vi "Event Handler.vi"(0 "Monkey in":refnum<class "Monkey.lvclass">, 5 "Event type":T1=enum."Message", 7 "Item Name":string, 9 "Data":variant, 11 "error in (no error)":errorcluster) -> (4 "Monkey out":refnum<class "Monkey.lvclass">, 15 "error out":errorcluster)   [LabVIEW 2020, in "Monkey.lvlib" / "Monkey.lvclass"]
doc: "This VI is the event handler of the uService: every time an event is triggered to the uService, this VI is called.\nNote: here you can access the Actor/Class data, but it will be the one coming out from Init. You cannot modify the values.\nThree different events are supported:\nI) Button Pressed: get called on a GUI button pressed. Item Name is the name (label) of the button, Data is empty.\nII) Shared Variable Updated: get called when a SV you subscribed to is updated. Item Name is the name of the SV, and Data is the value (note: you need to convert it to the proper type).\nIII) Message: get called every time a user event is generated using Send Message to Event Handler. The values of Item Name and Data are the one given to the Send Message to Event Handler.\nIV) Ready to launch?: this frame get called every time a new Run is initiated. Each uService is responsible of performing a self check before giving back the green light for the Run to start."
uses:
  Monkey.lvclass
  TALOS/TALOS_PPL.lvlibp/Father of all uServices/Father of all uServices/Event Handler Items.ctl
  Monkey Consumer Case Selector.ctl
  Run Utilities/TypeDefs/Messages/Schedule Message.ctl
  Run Utilities/TypeDefs/DAQ Control.ctl
  Run Utilities/Schedule/Schedule.lvclass
  Run Utilities/TypeDefs/Script Checker Result.ctl
  Inner stop message.ctl
  Run Utilities/Run Block/Run Block.lvclass
  TALOS/TALOS_PPL.lvlibp/Father of all uServices/Father of all uServices/Father of all uServices.lvclass
  Monkey.lvclass/Monkey.ctl
  Run Utilities/Run Utilities.lvlib
  TALOS/TALOS_PPL.lvlibp
  C:/LabVIEW Code/CIRCUS/TALOS/TALOS_PPL.lvlibp/Father of all uServices/Father of all uServices/Father of all uServices.lvclass
  C:/LabVIEW Code/CIRCUS/TALOS/TALOS_PPL.lvlibp/Ancestor/Ancestor/Ancestor.lvclass
  C:/LabVIEW Code/CIRCUS/TALOS/Actor Framework.lvlibp/1abvi3w/vi.lib/ActorFramework/Actor/Actor.lvclass
  C:/LabVIEW Code/CIRCUS/CIRCUS uServices et al/Monkey/Monkey.lvclass
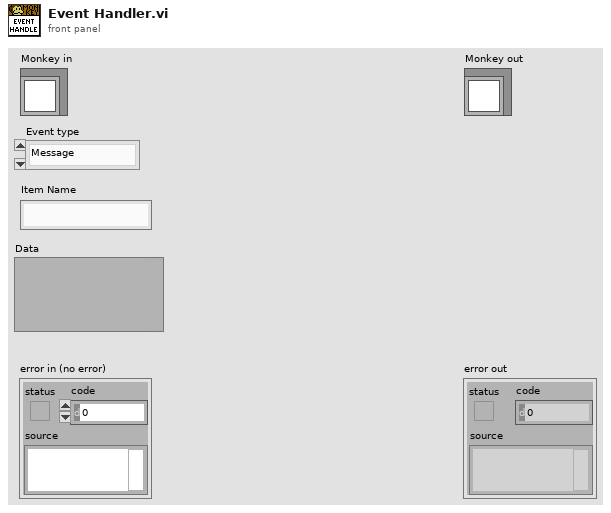
[diagram p1: front panel]
types:
  T1 = typedef "TALOS_PPL.lvlibp/Father of all uServices.lvlib/Father of all uServices.lvclass/Event Handler Items.ctl" = enum16{"Button Pressed", "Message", "Ready to launch?", "Safe Mode", "Start RUN", "Stop RUN"}
  T2 = typedef "Monkey.lvlib/Monkey.lvclass/Monkey Consumer Case Selector.ctl" = enum16{"Init", "Update GUI", "New schedule", "Check Script", "Submit Script", "Banana arrived", "Optimiser - evaluate RUN", "Optimiser - update RUN", "Quality Check", "What to do next", "Update Crit Lvl", "Skip Run", "Stop Schedule", "Skip schedule", "Append", "Update index", "Delete cell", "Move cell"}
  T3 = typedef "Run Utilities.lvlib/Schedule Message.ctl" = cluster{"uS Name":string, "Synchronised":bool, "DAQ Control":T4, "Schedule":refnum<class "Schedule.lvclass">, "Append to top?":bool}
  T4 = typedef "Run Utilities.lvlib/DAQ Control.ctl" = enum16{"On", "Off", "External"}
  T5 = typedef "Run Utilities.lvlib/Script Checker Result.ctl" = enum16{"Passed", "Failed", "Empty"}
  T6 = typedef "Monkey.lvlib/Monkey.lvclass/Inner stop message.ctl" = cluster{"Old value":bool, "Gracefully?":bool}
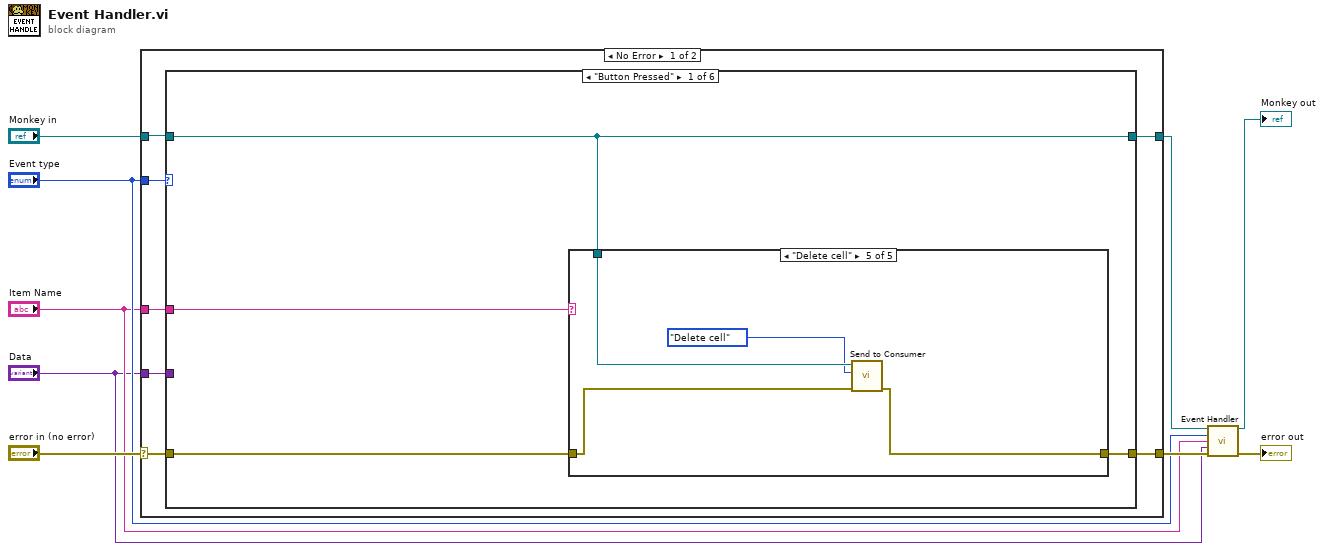
[diagram p0: block diagram]
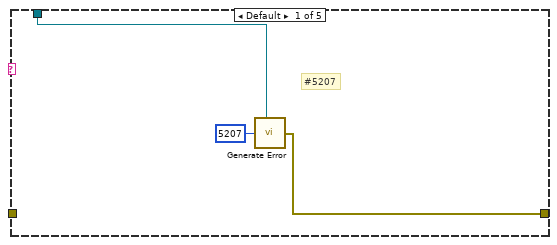
[diagram p2: hidden frame]
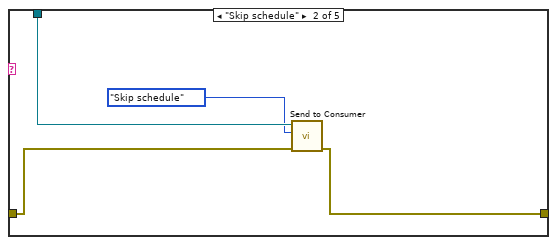
[diagram p3: hidden frame]
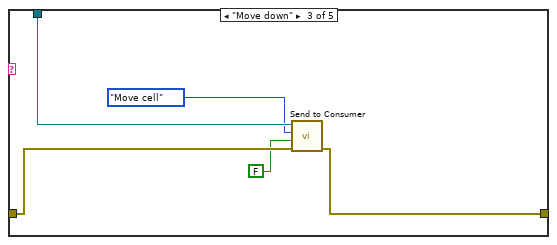
[diagram p4: hidden frame]
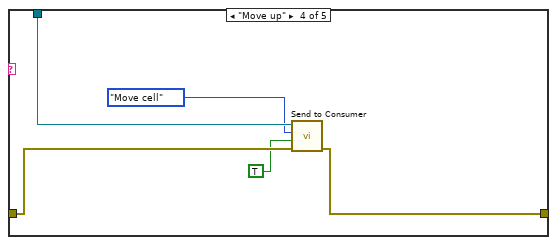
[diagram p5: hidden frame]
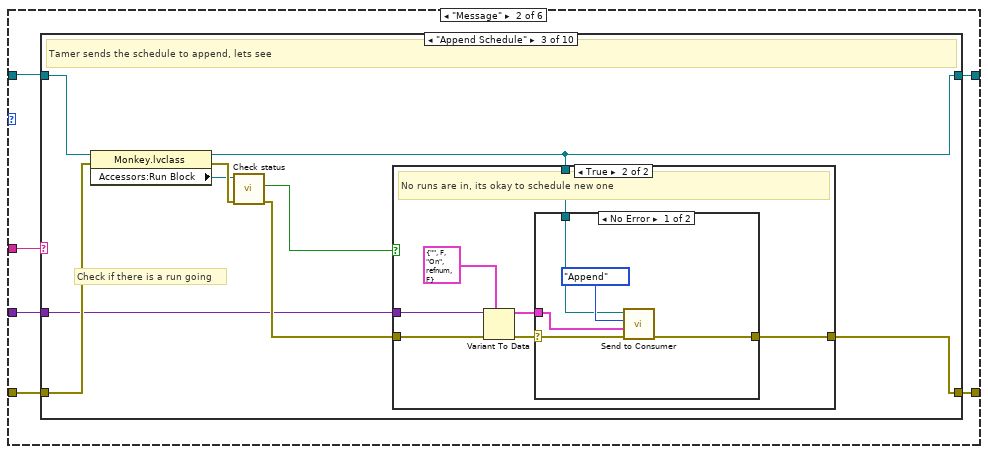
[diagram p6: hidden frame]
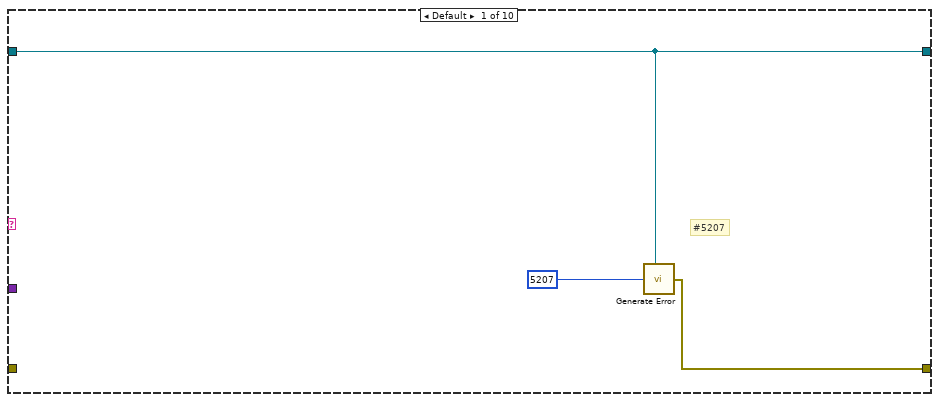
[diagram p7: hidden frame]
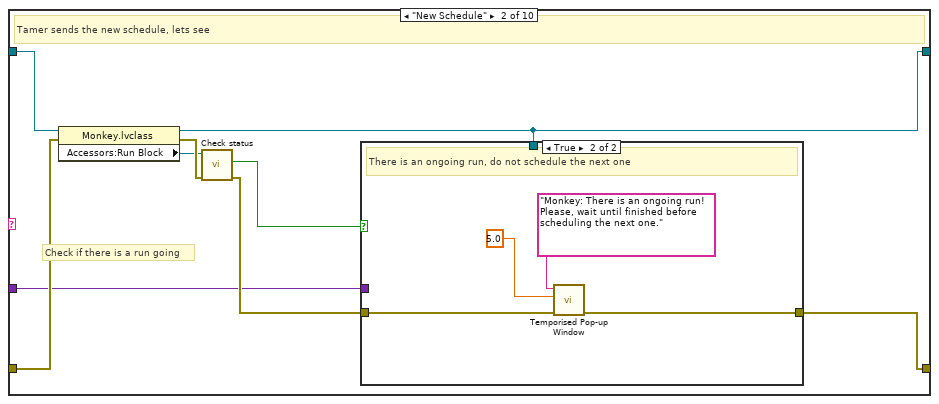
[diagram p8: hidden frame]
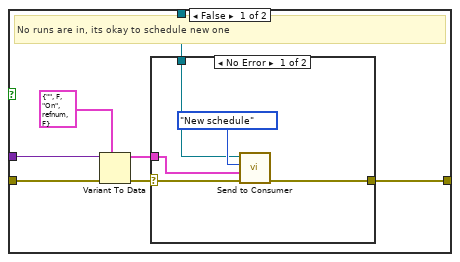
[diagram p9: hidden frame]
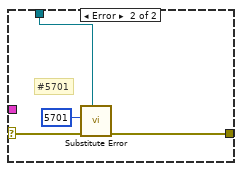
[diagram p10: hidden frame]
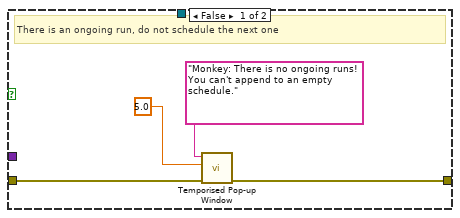
[diagram p11: hidden frame]
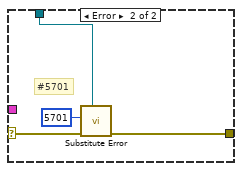
[diagram p12: hidden frame]
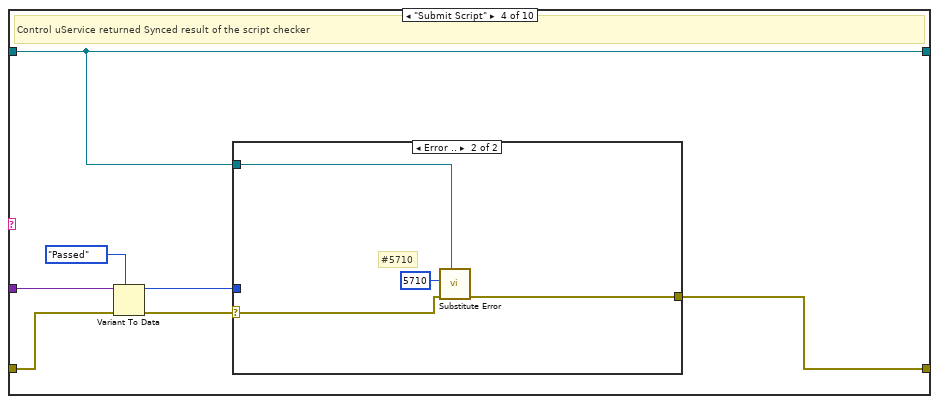
[diagram p13: hidden frame]
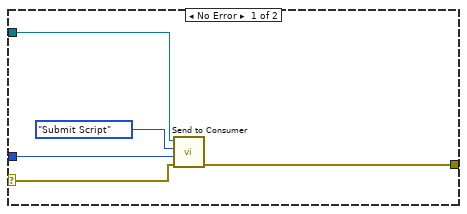
[diagram p14: hidden frame]
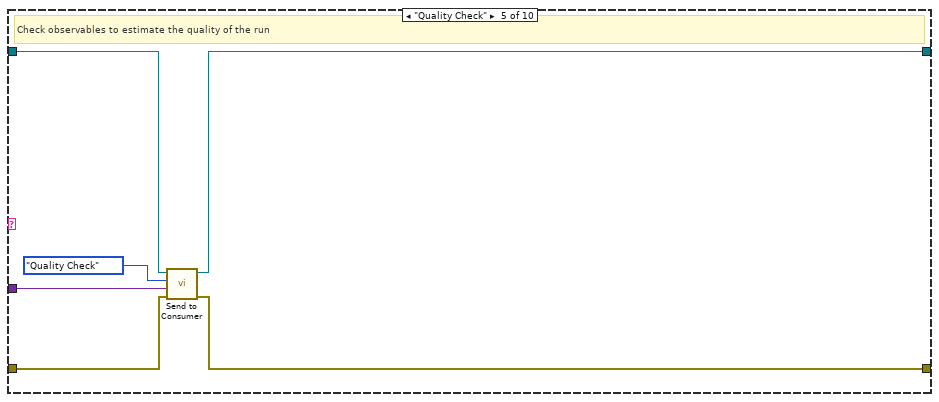
[diagram p15: hidden frame]
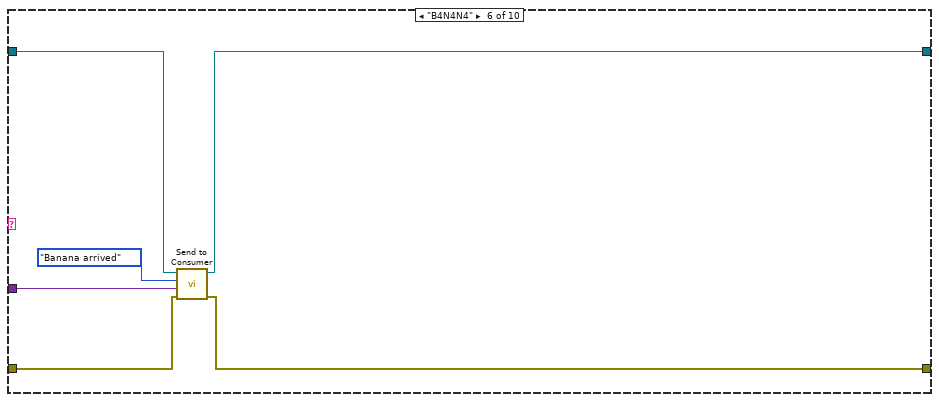
[diagram p16: hidden frame]
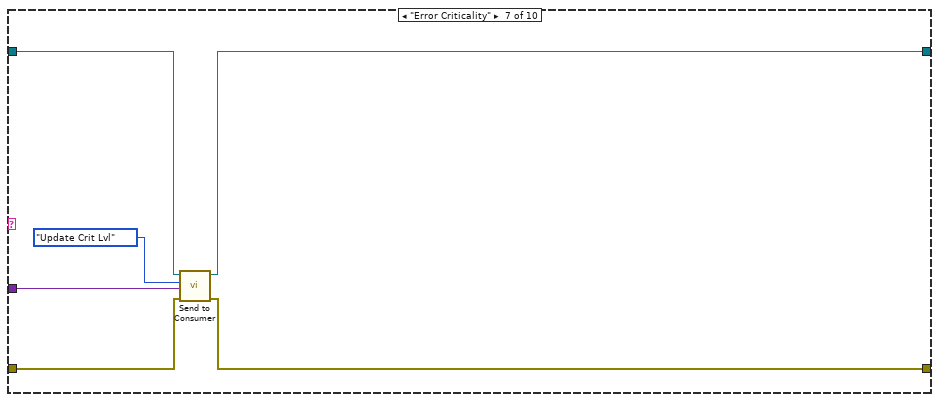
[diagram p17: hidden frame]
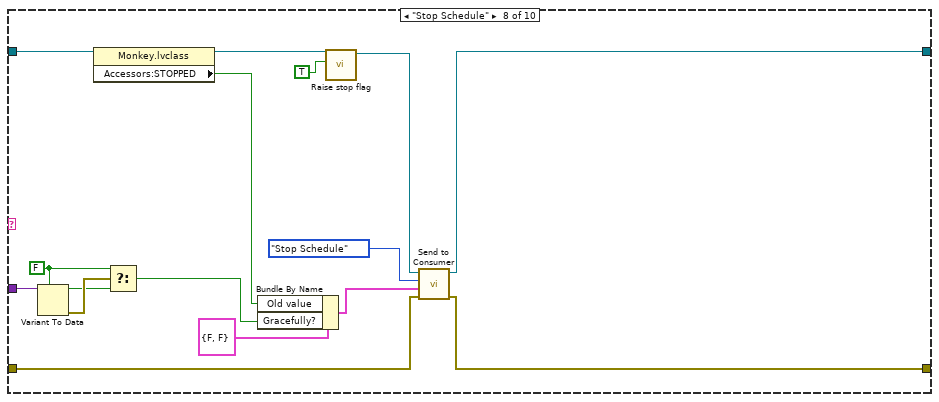
[diagram p18: hidden frame]
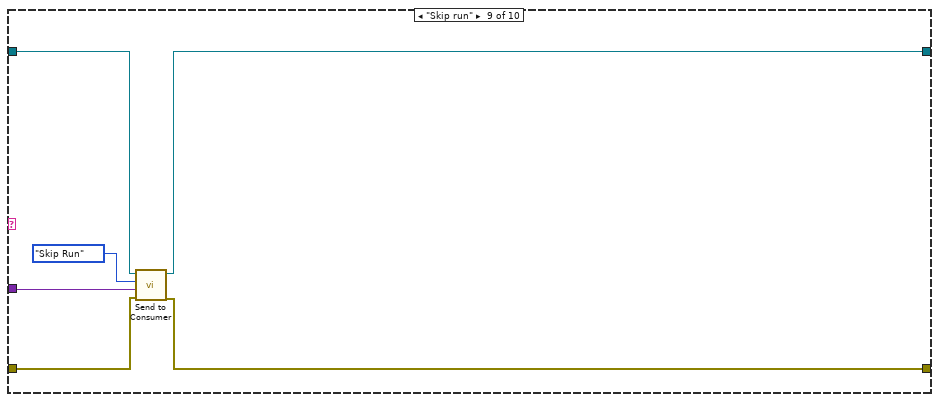
[diagram p19: hidden frame]
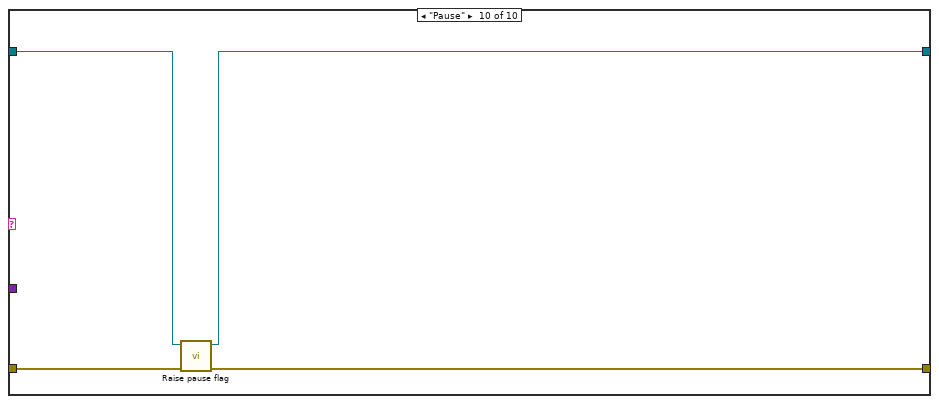
[diagram p20: hidden frame]
diagram:
  n1 = case shown="No Error" "error in (no error)" {
    selector: "error in (no error)" -> [w14 w198]
    tunnel: [w15 w198] -> w7
    tunnel: [w11 w197] -> w4
    tunnel: "Monkey in" -> [w10 w197]
    tunnel: "Event type" -> [w16 _]
    tunnel: "Item Name" -> [w13 _]
    tunnel: "Data" -> [w12 _]
    frame No Error {
      n2 = case shown="\"Button Pressed\"" w16 {
        tunnel: [w20 w43 w173 w182 w186 w193] -> w15
        tunnel: w14 -> [w18 w47 w174 w184 w189 w196]
        tunnel: w13 -> [w19 w46 _ _ _ _]
        tunnel: w10 -> [w17 w44 w172 w178 w190 w192]
        tunnel: w12 -> [_ w45 w170 _ _ _]
        tunnel: [w17 w42 w169 w180 w185 w191] -> w11
        frame "Button Pressed" {
          n3 = case shown="\"Delete cell\"" w19 {
            tunnel: w18 -> [_ w26 w31 w36 w40]
            tunnel: [w21 w25 w30 w35 w39] -> w20
            tunnel: w17 -> [w22 w27 w32 w37 w41]
            frame Default {
              # "#5207"
              n4 = call "Generate Error.vi"("Class"=w22, "Error Code"=5207) -> ("error out"=w21:errorcluster)  [unwired: 5 in]
            }
            frame "Skip schedule" {
              n5 = call "Send to Consumer.vi"("error in (no error)"=w26, "Case ID"=Monkey_Consumer_Case_Selector."Skip schedule" ("Monkey Consumer Case Selector"), "uService Template in"=w27) -> ("error out"=w25:errorcluster)  [unwired: 7 in, 1 out]
            }
            frame "Move down" {
              n6 = call "Send to Consumer.vi"("error in (no error)"=w31, "Data"=FALSE, "Case ID"=Monkey_Consumer_Case_Selector."Move cell" ("Monkey Consumer Case Selector"), "uService Template in"=w32) -> ("error out"=w30:errorcluster)  [unwired: 6 in, 1 out]
            }
            frame "Move up" {
              n7 = call "Send to Consumer.vi"("error in (no error)"=w36, "Data"=TRUE, "Case ID"=Monkey_Consumer_Case_Selector."Move cell" ("Monkey Consumer Case Selector"), "uService Template in"=w37) -> ("error out"=w35:errorcluster)  [unwired: 6 in, 1 out]
            }
            frame "Delete cell" {
              n8 = call "Send to Consumer.vi"("error in (no error)"=w40, "Case ID"=Monkey_Consumer_Case_Selector."Delete cell" ("Monkey Consumer Case Selector"), "uService Template in"=w41) -> ("error out"=w39:errorcluster)  [unwired: 7 in, 1 out]
            }
          }
        }
        frame "Message" {
          n9 = case shown="\"Append Schedule\"" w46 {
            tunnel: w47 -> [_ w59 w88 w114 w128 w135 w142 w158 w164 w167]
            tunnel: w45 -> [_ w56 w85 w115 w130 w133 w141 w149 w163 _]
            tunnel: w44 -> [w48 w52 w81 w109 w126 w132 w138 w155 w159 w168]
            tunnel: [w49 w55 w84 w110 w127 w134 w140 w157 w162 w166] -> w43
            tunnel: [w48 w51 w80 w109 w125 w131 w137 w154 w160 w165] -> w42
            frame Default {
              # "#5207"
              n10 = call "Generate Error.vi"("Class"=w48, "Error Code"=5207) -> ("error out"=w49:errorcluster)  [unwired: 5 in]
            }
            frame "New Schedule" {
              # "Check if there is a run going"
              # "Tamer sends the new schedule, lets see"
              n11 = property class="Monkey.lvclass"(reference=w52, error in=w59) -> (reference out=w51:refnum<class "Monkey.lvclass">, error out=w57:errorcluster, "Accessors:Run Block"=w54:refnum<class "Run Block.lvclass">)
              n12 = call-dynamic "Check status.vi"("error in (no error)"=w57, "Run Block in"=w54) -> ("error out"=w58:errorcluster, "Running"=w53:bool)  [unwired: 7 in, 1 out]
              n13 = case shown="True" w53 {
                tunnel: w56 -> [w66 _]
                tunnel: [w63 w76] -> w55
                tunnel: w51 -> [w62 _]
                tunnel: w58 -> [w61 w79]
                frame False {
                  # "No runs are in, its okay to schedule new one"
                  n14 = Variant To Data(error in=w61, type=T3 {"uS Name"="", "Synchronised"=FALSE, "DAQ Control"=enum."On", "Schedule"=refnum, "Append to top?"=FALSE} ("Monkey Schedule Message"), Variant=w66) -> (data=w64:T3, error out=w65:errorcluster)
                  n15 = case shown="No Error" w65 {
                    selector: w65 -> [w69 w75]
                    tunnel: w64 -> [w68 _]
                    tunnel: w62 -> [w70 w72]
                    tunnel: [w67 w73] -> w63
                    frame No Error {
                      n16 = call "Send to Consumer.vi"("error in (no error)"=w69, "Data"=w68, "Case ID"=Monkey_Consumer_Case_Selector."New schedule" ("Monkey Consumer Case Selector"), "uService Template in"=w70) -> ("error out"=w67:errorcluster)  [unwired: 6 in, 1 out]
                    }
                    frame Error {
                      # "#5701"
                      n17 = call "Substitute Error.vi"("LabVIEW Object"=w72, "error in (no error)"=w75, "Error Code"=5701) -> ("error out"=w73:errorcluster)  [unwired: 8 in]
                    }
                  }
                }
                frame True {
                  # "There is an ongoing run, do not schedule the next one"
                  n18 = call "Temporised Pop-up Window.vi"("error in (no error)"=w79, "Timeout"=5.0, "Text"="Monkey: There is an ongoing run! Please, wait until finished before scheduling the next one.") -> ("error out"=w76:errorcluster)  [unwired: 8 in]
                }
              }
            }
            frame "Append Schedule" {
              # "Check if there is a run going"
              # "Tamer sends the schedule to append, lets see"
              n19 = property class="Monkey.lvclass"(reference=w81, error in=w88) -> (reference out=w80:refnum<class "Monkey.lvclass">, error out=w86:errorcluster, "Accessors:Run Block"=w83:refnum<class "Run Block.lvclass">)
              n20 = call-dynamic "Check status.vi"("error in (no error)"=w86, "Run Block in"=w83) -> ("error out"=w87:errorcluster, "Running"=w82:bool)  [unwired: 7 in, 1 out]
              n21 = case shown="True" w82 {
                tunnel: w85 -> [_ w99]
                tunnel: [w89 w96] -> w84
                tunnel: w80 -> [_ w95]
                tunnel: w87 -> [w92 w94]
                frame False {
                  # "There is an ongoing run, do not schedule the next one"
                  n22 = call "Temporised Pop-up Window.vi"("error in (no error)"=w92, "Timeout"=5.0, "Text"="Monkey: There is no ongoing runs! You can't append to an empty schedule.") -> ("error out"=w89:errorcluster)  [unwired: 8 in]
                }
                frame True {
                  # "No runs are in, its okay to schedule new one"
                  n23 = Variant To Data(error in=w94, type=T3 {"uS Name"="", "Synchronised"=FALSE, "DAQ Control"=enum."On", "Schedule"=refnum, "Append to top?"=FALSE} ("Monkey Schedule Message"), Variant=w99) -> (data=w97:T3, error out=w98:errorcluster)
                  n24 = case shown="No Error" w98 {
                    selector: w98 -> [w102 w108]
                    tunnel: w97 -> [w101 _]
                    tunnel: w95 -> [w103 w105]
                    tunnel: [w100 w106] -> w96
                    frame No Error {
                      n25 = call "Send to Consumer.vi"("error in (no error)"=w102, "Data"=w101, "Case ID"=Monkey_Consumer_Case_Selector."Append" ("Monkey Consumer Case Selector"), "uService Template in"=w103) -> ("error out"=w100:errorcluster)  [unwired: 6 in, 1 out]
                    }
                    frame Error {
                      # "#5701"
                      n26 = call "Substitute Error.vi"("LabVIEW Object"=w105, "error in (no error)"=w108, "Error Code"=5701) -> ("error out"=w106:errorcluster)  [unwired: 8 in]
                    }
                  }
                }
              }
            }
            frame "Submit Script" {
              # "Control uService returned Synced result of the script checker"
              n27 = Variant To Data(error in=w114, type=Script_Checker_Result."Passed" ("Script Checker Result"), Variant=w115) -> (data=w111:T5, error out=w112:errorcluster)
              n28 = case shown="Error .." w112 {
                selector: w112 -> [w117 w122]
                tunnel: w111 -> [w119 _]
                tunnel: w109 -> [w118 w123]
                tunnel: [w116 w124] -> w110
                frame No Error {
                  n29 = call "Send to Consumer.vi"("error in (no error)"=w117, "Data"=w119, "Case ID"=Monkey_Consumer_Case_Selector."Submit Script" ("Monkey Consumer Case Selector"), "uService Template in"=w118) -> ("error out"=w116:errorcluster)  [unwired: 6 in, 1 out]
                }
                frame Error {
                  # "#5710"
                  n30 = call "Substitute Error.vi"("LabVIEW Object"=w123, "error in (no error)"=w122, "Error Code"=5710) -> ("error out"=w124:errorcluster)  [unwired: 8 in]
                }
              }
            }
            frame "Quality Check" {
              # "Check observables to estimate the quality of the run"
              n31 = call "Send to Consumer.vi"("error in (no error)"=w128, "Data"=w130, "Case ID"=Monkey_Consumer_Case_Selector."Quality Check" ("Monkey Consumer Case Selector"), "uService Template in"=w126) -> ("error out"=w127:errorcluster, "uService Template out"=w125:refnum<class "Monkey.lvclass">)  [unwired: 6 in]
            }
            frame "B4N4N4" {
              n32 = call "Send to Consumer.vi"("error in (no error)"=w135, "Data"=w133, "Case ID"=Monkey_Consumer_Case_Selector."Banana arrived" ("Monkey Consumer Case Selector"), "uService Template in"=w132) -> ("error out"=w134:errorcluster, "uService Template out"=w131:refnum<class "Monkey.lvclass">)  [unwired: 6 in]
            }
            frame "Error Criticality" {
              n33 = call "Send to Consumer.vi"("error in (no error)"=w142, "Data"=w141, "Case ID"=Monkey_Consumer_Case_Selector."Update Crit Lvl" ("Monkey Consumer Case Selector"), "uService Template in"=w138) -> ("error out"=w140:errorcluster, "uService Template out"=w137:refnum<class "Monkey.lvclass">)  [unwired: 6 in]
            }
            frame "Stop Schedule" {
              w150 = FALSE
              n34 = Variant To Data(type=w150, Variant=w149) -> (data=w151:bool, error out=w152:errorcluster)  [unwired: 1 in]
              n35 = property class="Monkey.lvclass"(reference=w155) -> (reference out=w145:refnum<class "Monkey.lvclass">, "Accessors:STOPPED"=w147:bool)  [unwired: 1 in, 1 out]
              n36 = Select(t=w150, s=w152, f=w151) -> (s? t:f=w148:bool)
              n37 = Bundle By Name(cluster=T6 {"Old value"=FALSE, "Gracefully?"=FALSE} ("Stop msg"), "Old value"=w147, "Gracefully?"=w148) -> (w146:T6)
              n38 = call-dynamic "Raise stop flag.vi"("on/off"=TRUE, "Monkey in"=w145) -> ("Monkey out"=w144:refnum<class "Monkey.lvclass">)  [unwired: 8 in, 1 out]
              n39 = call "Send to Consumer.vi"("error in (no error)"=w158, "Data"=w146, "Case ID"=Monkey_Consumer_Case_Selector."Stop Schedule" ("Monkey Consumer Case Selector"), "uService Template in"=w144) -> ("error out"=w157:errorcluster, "uService Template out"=w154:refnum<class "Monkey.lvclass">)  [unwired: 6 in]
            }
            frame "Skip run" {
              n40 = call "Send to Consumer.vi"("error in (no error)"=w164, "Data"=w163, "Case ID"=Monkey_Consumer_Case_Selector."Skip Run" ("Monkey Consumer Case Selector"), "uService Template in"=w159) -> ("error out"=w162:errorcluster, "uService Template out"=w160:refnum<class "Monkey.lvclass">)  [unwired: 6 in]
            }
            frame "Pause" {
              n41 = call-dynamic "Raise pause flag.vi"("error in (no error)"=w167, "Monkey in"=w168) -> ("error out"=w166:errorcluster, "Monkey out"=w165:refnum<class "Monkey.lvclass">)  [unwired: 8 in]
            }
          }
        }
        frame "Ready to launch?" {
          # "Don't remove this wire!"
          # "Just give green light: \"Cogito ergo sum\" - Volpe"
          n42 = call-dynamic "Go-NoGo.vi"("error in (no error)"=w174, "Go-NoGo Data"=w170, "Go?"=TRUE, "Father of all uServices in"=w172) -> ("error out"=w173:errorcluster, "Father of all uServices out"=w169:refnum<class "Monkey.lvclass">)  [unwired: 6 in]
        }
        frame "Safe Mode" {
          n43 = property class="Monkey.lvclass"(reference=w178) -> (reference out=w177:refnum<class "Monkey.lvclass">, "Accessors:STOPPED"=w176:bool)  [unwired: 1 in, 1 out]
          n44 = Bundle By Name(cluster=T6 {"Old value"=FALSE, "Gracefully?"=FALSE} ("Stop msg"), "Old value"=w176) -> (w175:T6)
          n45 = call "Send to Consumer.vi"("Data"=w175, "Case ID"=Monkey_Consumer_Case_Selector."Stop Schedule" ("Monkey Consumer Case Selector"), "uService Template in"=w177) -> ("error out"=w181:errorcluster, "uService Template out"=w180:refnum<class "Monkey.lvclass">)  [unwired: 7 in]
          n46 = Merge Errors(w181, w184) -> (w182:errorcluster)
        }
        frame "Start RUN" {
          n47 = call "Update GUI.vi"("error in (no error)"=w189, "Data"="Experiment running!" ("GUI Item Name"), "GUI Item Name"="Current Action", "uService Template in"=w190) -> ("error out"=w186:errorcluster, "uService Template out"=w185:refnum<class "Monkey.lvclass">)  [unwired: 6 in]
        }
        frame "Stop RUN" {
          n48 = call "Update GUI.vi"("error in (no error)"=w196, "Data"="Experiment finished! Ending the script..." ("GUI Item Name"), "GUI Item Name"="Current Action", "uService Template in"=w192) -> ("error out"=w193:errorcluster, "uService Template out"=w191:refnum<class "Monkey.lvclass">)  [unwired: 6 in]
        }
      }
    }
    frame Error {
    }
  }
  n49 = call-parent "Event Handler.vi"("uService Template in"=w4, "Event type"="Event type", "Item Name"="Item Name", "Data"="Data", "error in (no error)"=w7) -> ("uService Template out"=→"Monkey out":refnum<class "Monkey.lvclass">, "error out"=→"error out":errorcluster)  [unwired: 9 in]
